vi "Format Data for ANSI-Export.vi"(7 "LT.Data.Languages":cluster{"ANSI":string[], "Unicode":string[]}, 11 "Translations":T1[](array[typedef])) -> (3 "ANSI string":string)   [LabVIEW 2019, in "Language Editor.lvlib"]
doc: "- - -\nCopyright (c) 2026, Merecs Engineering GmbH"
uses:
  Language Editor.lvlib
  Language Selection/TypeDefs/Cluster Language.ctl
  Language Selection/TypeDefs/Cluster PropertyTranslation.ctl
  Language Selection/TypeDefs/Enum Property Type.ctl
  Language Selection/Language Selection.lvlib
panel:
  # "Connector Pane"
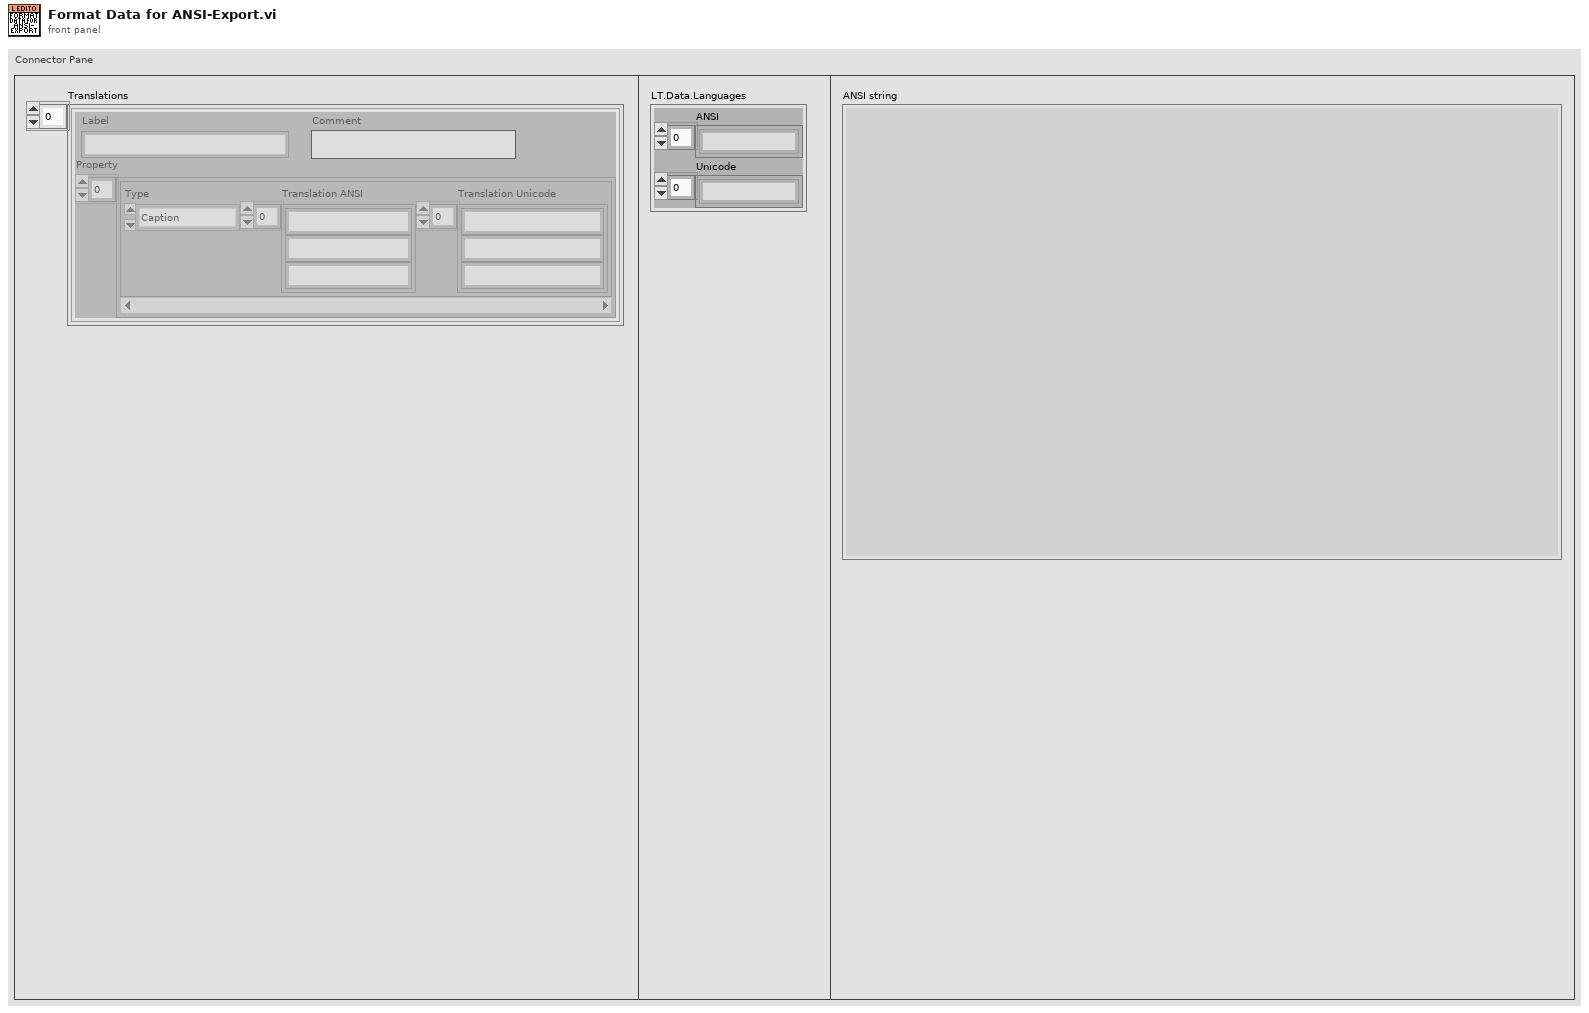
[diagram p1: front panel]
types:
  T1 = typedef "Language Selection.lvlib/Cluster Language.ctl" = cluster{"Label":string, "Comment":string, "Property":T2[]}
  T2 = typedef "Language Selection.lvlib/Cluster PropertyTranslation.ctl" = cluster{"Type":T3, "Translation ANSI":string[], "Translation Unicode":string[]}
  T3 = typedef "Language Selection.lvlib/Enum Property Type.ctl" = enum16{"NA", "Caption", "String Value", "Boolean Text", "Ring Strings", "1D Array Elements", "2D Array Elements", "(MC)Listbox Header", "(MC)Listbox Items", "Tab Pages Names", "X & Y GraphChart", "Plot Names", "Table Headers", "Table Items", "TipStrip", "Combobox Strings", "Cursor Name", "Tree Col Headers"}
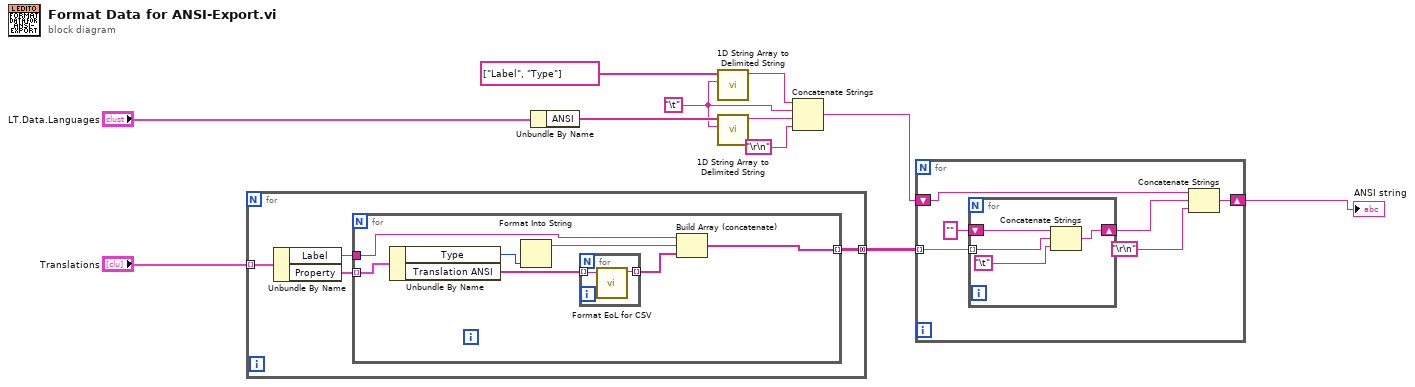
[diagram p0: block diagram]
diagram:
  w7 = "\t"
  n1 = for {
    tunnel: "Translations" -> [w15] mode=indexing
    tunnel: [w12] -> w6 mode=concatenating
    n2 = Unbundle By Name(w15) -> ("Label"=w13:string, "Property"=w14:T2[])
    n3 = for {
      tunnel: w14 -> [w22] mode=indexing
      tunnel: w13 -> [w19]
      tunnel: [w16] -> w12 mode=indexing
      n4 = Unbundle By Name(w22) -> ("Type"=w21:T3, "Translation ANSI"=w18:string[])
      n5 = Format Into String(w21) -> (resulting string=w20:string)  [unwired: 3 in, 1 out]
      n6 = for {
        tunnel: w18 -> [w24] mode=indexing
        tunnel: [w23] -> w17 mode=indexing
        n7 = call "Format EoL for CSV.vi"("String In"=w24) -> ("String"=w23:string)  [unwired: 10 in]
      }
      n8 = Build Array (concatenate)(w19, w20, w17) -> (w16:string[])
    }
  }
  n9 = Unbundle By Name("LT.Data.Languages") -> ("ANSI"=w10:string[])
  n10 = call <vilib>:"1D String Array to Delimited String.vi"("delimiter"=w7, "string array"=string[] ["Label", "Type"] ("new element/subarray")) -> ("delimited string"=w9:string)  [unwired: 9 in]
  n11 = call <vilib>:"1D String Array to Delimited String.vi"("delimiter"=w7, "string array"=w10) -> ("delimited string"=w8:string)  [unwired: 9 in]
  n12 = Concatenate Strings(w9, w7, w8, "\r\n") -> (w5:string)
  n13 = for {
    tunnel: w6 -> [w30] mode=indexing
    shift-right: [w27] -> w1
    shift-left: w5 -> [w28]
    n14 = for {
      shift-right: [w32] -> w29
      shift-left: "" ("string") -> [w34]
      tunnel: w30 -> [w33] mode=indexing
      n15 = Concatenate Strings(w34, w33, "\t") -> (w32:string)
    }
    n16 = Concatenate Strings(w28, w29, "\r\n") -> (w27:string)
  }
  "ANSI string" <- w1
